vi "LTE Change Band Status.vi"(8 "error in (no error)":errorcluster caption="에러 입력(에러 없음)", 9 "BandWidth":T1, 10 "UL Channel":i32, 11 "Instrument Manager 입력":refnum<class "Instrument Manager.lvclass">) -> (0 "error out":errorcluster caption="에러 출력", 3 "Instrument Manager 출력":refnum<class "Instrument Manager.lvclass">)   [LabVIEW 2023, in "Instrument Manager.lvclass"]
uses:
  Instrument Manager.lvclass
  Instrument Manager.lvclass/Instrument Manager.ctl
  Module/ANRITSU Call Box/Type Definition/LTE Supported BandWidth.ctl
  Module/ANRITSU Call Box/ANRITSU Call Box.lvlib
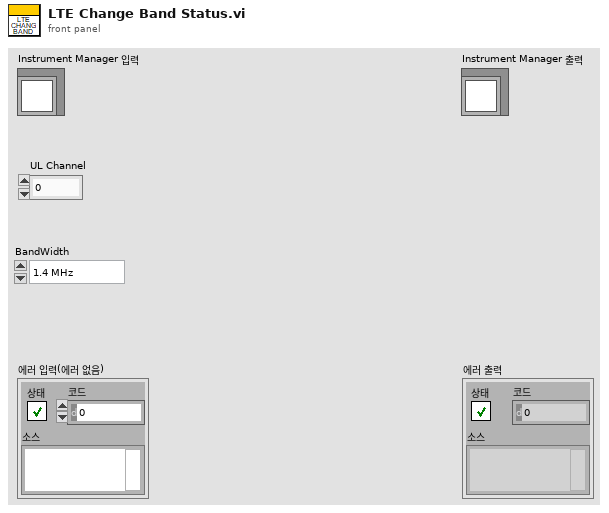
[diagram p1: front panel]
types:
  T1 = typedef "ANRITSU Call Box.lvlib/LTE Supported BandWidth.ctl" = enum16{"1.4 MHz", "3 MHz", "5 MHz", "10 MHz", "15 MHz", "20 MHz"}
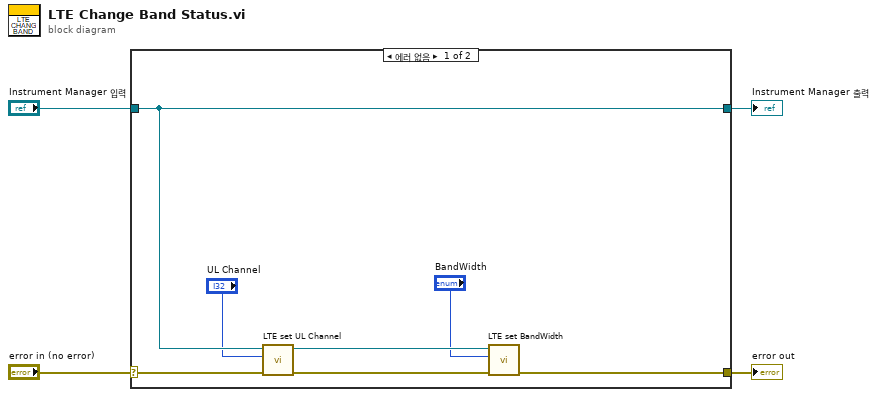
[diagram p0: block diagram]
diagram:
  n1 = case shown="에러 없음" "error in (no error)" {
    selector: "error in (no error)" -> [w11 w13]
    tunnel: [w9 w13] -> w3
    tunnel: [w8 w12] -> w1
    tunnel: "Instrument Manager 입력" -> [w8 w12]
    frame No Error {
      n2 = call "LTE set UL Channel.vi"("error in (no error)"=w11, "UL Channel"="UL Channel", "Instrument Manager 입력"=w8) -> ("error out"=w10:errorcluster, "Instrument Manager 출력"=w7:refnum<class "Instrument Manager.lvclass">)  [unwired: 7 in]
      n3 = call "LTE set BandWidth.vi"("error in (no error)"=w10, "BandWidth"="BandWidth", "Instrument Manager 입력"=w7) -> ("error out"=w9:errorcluster)  [unwired: 7 in, 1 out]
    }
    frame Error {
    }
  }
  "error out" <- w3
  "Instrument Manager 출력" <- w1
